vi "ToTable.vi"(8 "error in":errorcluster, 9 "Table Index (0)":i32, 10 "variant":variant, 11 "Shared Memory editor node in":refnum<class "Shared Memory editor node.lvclass">) -> (0 "error out":errorcluster, 1 "row headers":string[](array[string]), 2 "table":string[][](array[string]), 3 "Shared Memory editor node out":refnum<class "Shared Memory editor node.lvclass">)   [LabVIEW 2014, in "Shared Memory editor node.lvclass"]
doc: "Generates the strings needed to display on a table based on the information found in the engine and module configuration classes."
uses:
  Shared Memory editor node.lvclass
  module/configuration/Shared Memory configuration.lvclass
  <vilib>/NI/Module Execution Interface/Engine Configuration/engine configuration.lvclass
  module/configuration/Shared Memory configuration.lvclass/Shared Memory configuration.ctl
  <vilib>/NI/Configuration Framework/serializable configuration/NISE_CEF_serializable configuration.lvclass/NISE_CEF_serializable configuration.ctl
  <vilib>/NI/Tag Bus/tag/tag descriptor.lvclass/tag descriptor.ctl
  <vilib>/NI/Tag Bus Module Framework/channel/TBM channel.lvclass/TBM channel.ctl
  module/configuration/Read Lines.vi
  <vilib>/Utility/LVClass/Get LV Class Name.vi
  <vilib>/NI/Configuration Framework/error generator/NISE_error generator.vi
  <vilib>/NI/Tag Bus Module Framework/channel/TBM channel.lvclass
  <vilib>/NI/Tag Bus/tag/tag descriptor.lvclass
  <vilib>/NI/Configuration Framework/serializable configuration/NISE_CEF_serializable configuration.lvclass
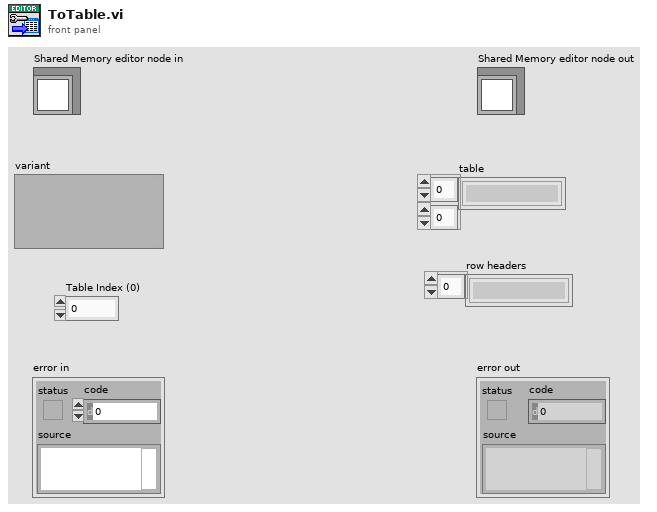
[diagram p1: front panel]
types:
  T1 = typedef "tag bus configurable plugin module configuration.lvclass/Line.ctl" = cluster{"channel":refnum<class "TBM channel.lvclass">}
  T2 = typedef "TBM channel.lvclass/channel classification.ctl" = enum16{"input data", "output data", "processing parameter", "processing result"}
  T3 = typedef "tag bus.lvlib/tag descriptor.lvclass/Data Type.ctl" = enum16{"Double", "Single", "I64", "I32", "I16", "I8", "U64", "U32", "U16", "U8", "Boolean", "String", "Array of Double", "Array of Single", "Array of I64", "Array of I32", "Array of I16", "Array of I8", "Array of U64", "Array of U32", "Array of U16", "Array of U8", "Array of Boolean", "Array of String"}
  T4 = typedef "Shared Memory editor node.lvclass/permissions.ctl" = enum32{"Write to Memory", "Read from Memory"}
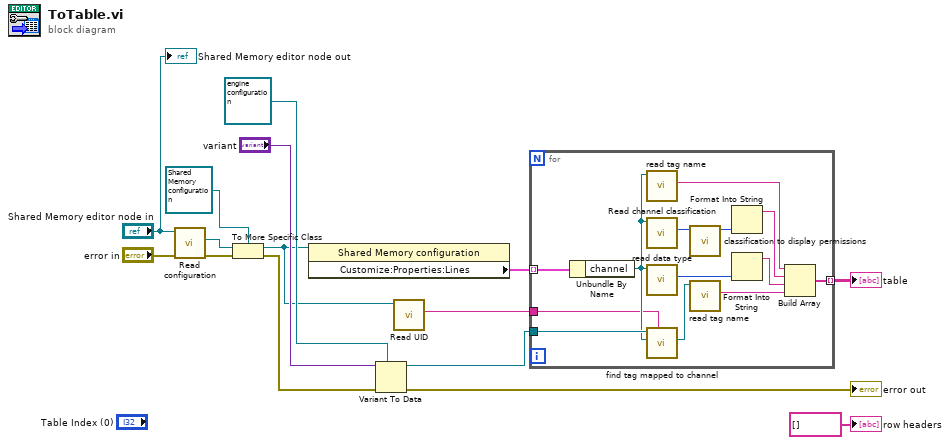
[diagram p0: block diagram]
diagram:
  n1 = call-dynamic "Read configuration.vi"("error in"="error in", "Shared Memory editor node in"="Shared Memory editor node in") -> ("error out"=w15:errorcluster, "configuration"=w6:refnum<class "NISE_CEF_serializable configuration.lvclass">)  [unwired: 7 in, 1 out]
  n2 = To More Specific Class(target class=refnum<class "Shared Memory configuration.lvclass"> refnum ("tag bus configurable plugin module configuration"), reference=w6, error in=w15) -> (specific class reference=w5:refnum<class "Shared Memory configuration.lvclass">, error out=w3:errorcluster)
  n3 = property class="Shared Memory configuration"(reference=w5) -> ("Customize:Properties:Lines"=w12:T1[])  [unwired: 1 in, 2 out]
  n4 = Variant To Data(error in=w3, type=refnum<class "engine configuration.lvclass"> refnum ("engine configuration"), Variant="variant") -> (data=w9:refnum<class "engine configuration.lvclass">, error out=→"error out":errorcluster)
  n5 = call <vilib>:"Read UID.vi"("configuration in"=w5) -> ("instance id"=w4:string)  [unwired: 8 in, 2 out]
  n6 = for {
    tunnel: w12 -> [w28] mode=indexing
    tunnel: w9 -> [w26]
    tunnel: [w17] -> w7 mode=indexing
    tunnel: w4 -> [w16]
    n7 = Unbundle By Name(w28) -> ("channel"=w20:refnum<class "TBM channel.lvclass">)
    n8 = call <vilib>:"read tag name.vi"("system tag in"=w20) -> ("name"=w27:string)  [unwired: 8 in, 2 out]
    n9 = call <vilib>:"Read channel classification.vi"("channel in"=w20) -> ("channel classification"=w24:T2)  [unwired: 8 in, 2 out]
    n10 = call <vilib>:"read data type.vi"("system tag in"=w20) -> ("data type"=w19:T3)  [unwired: 8 in, 2 out]
    n11 = call <vilib>:"find tag mapped to channel.vi"("owner"=w16, "channel"=w20, "engine configuration in"=w26) -> ("tag"=w25:refnum<class "tag descriptor.lvclass">)  [unwired: 6 in, 2 out]
    n12 = call "classification to display permissions.vi"("channel classification"=w24) -> ("permissions"=w23:T4)  [unwired: 10 in]
    n13 = call <vilib>:"read tag name.vi"("system tag in"=w25) -> ("name"=w21:string)  [unwired: 8 in, 2 out]
    n14 = Format Into String(w23) -> (resulting string=w22:string)  [unwired: 3 in, 1 out]
    n15 = Format Into String(w19) -> (resulting string=w18:string)  [unwired: 3 in, 1 out]
    n16 = Build Array(w27, w22, w18, w21) -> (w17:string[])
  }
  "table" <- w7
  "Shared Memory editor node out" <- "Shared Memory editor node in"
  "row headers" <- string[] [] ("row headers")
